vi "Create Synchronized Palette.vi"(6 "Exclude Dir Name pattern":string="^_", 7 "Palette Icon":picture, 8 "error in":errorcluster, 9 "Recursively (F)":bool, 10 "Folder Path":path, 11 "Palette File Path (empty)":path) -> (0 "error out":errorcluster, 2 "All Palette File Paths":path[](array[path]), 3 "Palette File Path out":path)   [LabVIEW 2014, in "VIHelpeksAPI.lvlib"]
doc: "The VI creates a palette file synchronized with the given folder. In addition, if enabled, the VI creates a synchronized palette in every sub-folder beneath the given folder recursively.\n\n<b>Palette icons</b>\nFor the given folder and all sub-folders beneath it (if enabled by <b>Recursively</b>), the VI looks for an image file to use as an icon for the respective palette. A folder's icon file can be one of the following:\n(1) A file with the same name as the folder and a <b>.png</b> extension that resides in the folder's parent directory.\n(2) A file with the <b>dir_icon.png</b> name that resides inside the folder itself.\nIf neither of these icon files is found, a default icon is applied to the respective palette.\nThe icon of the top-level palette can be defined explicitly in the <b>Palette Icon</b> input terminal.\n\n\n::: VI Helpeks :::\nCopyright (c) 2000-2026 Konstantin Shifershteyn. All rights reserved."
uses:
  VIHelpeksAPI.lvlib
  <vilib>/Palette API/Palette Menu/Public Type Define/Palette type.ctl
  <vilib>/Palette API/Palette Menu/Public Type Define/View Format.ctl
  <vilib>/Palette API/Palette Menu/Public Type Define/Palette Data.ctl
  <vilib>/Palette API/Palette Menu/Public Type Define/Items.ctl
  <vilib>/Palette API/Palette Menu/Public Type Define/Item.ctl
  <vilib>/Palette API/Palette Menu/Public Type Define/Help Info.ctl
  <vilib>/Palette API/Palette Menu/Public Type Define/Synchronize Info.ctl
  <vilib>/Palette API/Palette Menu/Palette Menu.lvlib
panel:
  # "VI Helpeks\nCopyright (c) 2012-2026 Konstantin Shifershteyn"
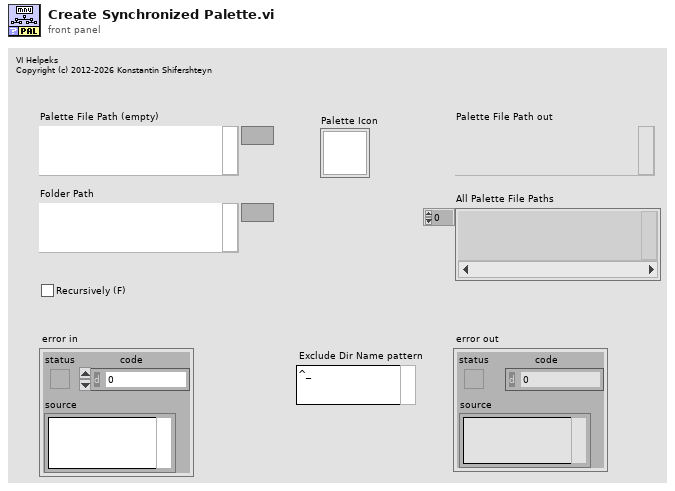
[diagram p1: front panel]
types:
  T1 = typedef "Palette Menu.lvlib/Palette Data.ctl" = cluster{"display name":string, "view format":T2, "palette width":i16, "items":T3, "256 color icon":picture, "B&W color icon":picture, "help information":T5, "palette description":string, "synchronize information":T6}
  T2 = typedef "Palette Menu.lvlib/View Format.ctl" = u16
  T3 = typedef "Palette Menu.lvlib/Items.ctl" = T4[]
  T4 = typedef "Palette Menu.lvlib/Item.ctl" = cluster{"item path":path, "library path (.lvlib)":path, "use default lvlib palette":bool, "short name":string, "place VI contents":bool, "hide synchronized item":bool, "reserve spot for synch item":bool, "configure when placing VI contents":bool}
  T5 = typedef "Palette Menu.lvlib/Help Info.ctl" = cluster{"help tag":string, "help file path ":path}
  T6 = typedef "Palette Menu.lvlib/Synchronize Info.ctl" = cluster{"synchronize with directory":bool, "synchronize directory path":path}
  T7 = typedef "Palette Menu.lvlib/Palette type.ctl" = i32
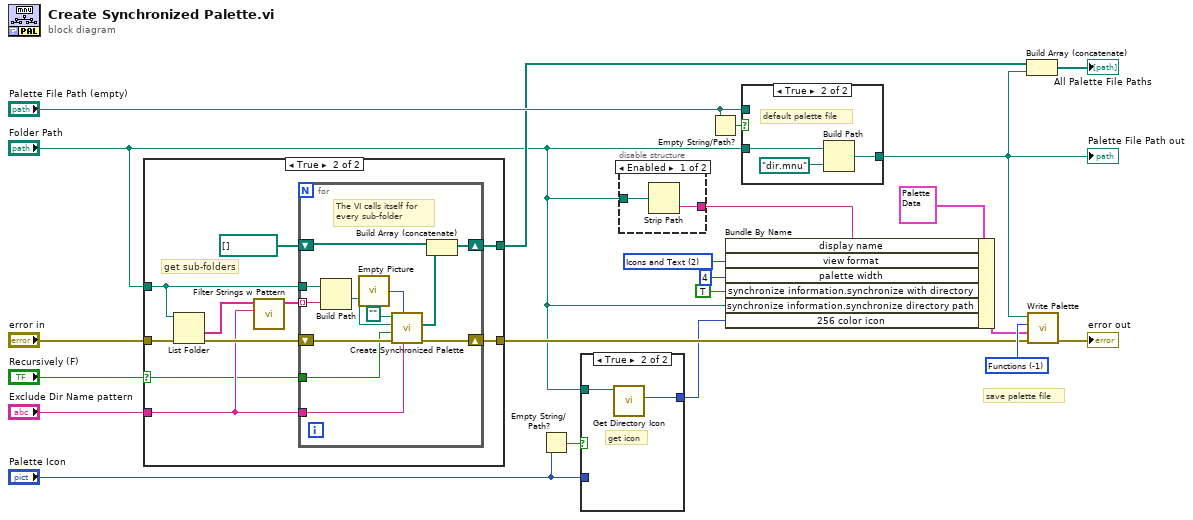
[diagram p0: block diagram]
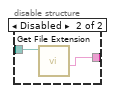
[diagram p5: hidden frame]
diagram:
  w19 = T2 2 items=["Icons", "Text", "Icons and Text"] ("view format")
  w18 = T7 -1 items=["Functions"=-1, "Controls"=-2] ("palette type")
  # "save palette file"
  n1 = case shown="True" "Recursively (F)" {
    selector: "Recursively (F)" -> [_ w25]
    tunnel: "error in" -> [w22 w32]
    tunnel: [w22 w29] -> w15
    tunnel: "Exclude Dir Name pattern" -> [_ w26]
    tunnel: "Folder Path" -> [_ w27]
    tunnel: [_ w23] -> w7
    frame False {
    }
    frame True {
      # "get sub-folders"
      n2 = List Folder(path=w27, error in=w32) -> (folder names=w31:string[], error out=w30:errorcluster)  [unwired: 2 in, 2 out]
      n3 = call "Filter Strings w Pattern.vi"("Exclude pattern(s) (^_)"=w26, "Array in"=w31) -> ("Array out"=w28:string[])  [unwired: 9 in]
      n4 = for {
        tunnel: w27 -> [w44]
        tunnel: w28 -> [w41] mode=indexing
        shift-right: [w42] -> w29
        shift-left: w30 -> [w43]
        tunnel: w26 -> [w40]
        tunnel: w25 -> [w39]
        shift-right: [w34] -> w23
        shift-left: path[] [] -> [w35]
        # "The VI calls itself for\nevery sub-folder"
        n5 = Build Path(base path=w44, name or relative path=w41) -> (appended path=w38:path)
        n6 = call "Empty Picture"() -> ("empty picture"=w33:picture)
        n7 = call "Create Synchronized Palette.vi"("Exclude Dir Name pattern"=w40, "Palette Icon"=w33, "error in"=w43, "Recursively (F)"=w39, "Folder Path"=w38, "Palette File Path (empty)"=path "") -> ("error out"=w42:errorcluster, "All Palette File Paths"=w36:path[])  [unwired: 3 in, 1 out]
        n8 = Build Array (concatenate)(w35, w36) -> (w34:path[])
      }
    }
  }
  n9 = Empty String/Path?(string/path="Palette Icon") -> (empty?=w3:bool)
  n10 = case shown="True" w3 {
    tunnel: [w45 w47] -> w1
    tunnel: "Folder Path" -> [_ w46]
    tunnel: "Palette Icon" -> [w45 _]
    frame False {
    }
    frame True {
      # "get icon"
      n11 = call "Get Directory Icon.vi"("Directory Path"=w46) -> ("Icon"=w47:picture)  [unwired: 8 in, 2 out]
    }
  }
  n12 = disable-structure shown="Enabled" {
    disable-tunnel: "Folder Path" -> [w49 w51]
    disable-tunnel: [w48 w50] -> w20
    frame Enabled {
      n13 = Strip Path(path=w49) -> (name=w48:string)  [unwired: 1 out]
    }
    frame Disabled {
      n14 = call <vilib>:"Get File Extension.vi"("file"=w51) -> ("filename without extension"=w50:string)  [unwired: 7 in, 3 out]
    }
  }
  n15 = Empty String/Path?(string/path="Palette File Path (empty)") -> (empty?=w9:bool)
  n16 = Bundle By Name(cluster=T1 {"display name"="", "view format"=2, "palette width"=4, "items"=[], "256 color icon"=bytes[0], "B&W color icon"=bytes[0], "help information"={"help tag"="", "help file path "=path ""}, "palette description"="", "synchronize information"={"synchronize with directory"=FALSE, "synchronize directory path"=path ""}} ("palette data"), "display name"=w20, "view format"=w19, "palette width"=i16 4, "synchronize information.synchronize with directory"=TRUE, "synchronize information.synchronize directory path"="Folder Path", "256 color icon"=w1) -> (w17:T1)
  n17 = case shown="True" w9 {
    tunnel: [w52 w54] -> w6
    tunnel: "Folder Path" -> [_ w53]
    tunnel: "Palette File Path (empty)" -> [w52 _]
    frame False {
    }
    frame True {
      # "default palette file"
      n18 = Build Path(base path=w53, name or relative path=path "dir.mnu") -> (appended path=w54:path)
    }
  }
  "Palette File Path out" <- w6
  n19 = Build Array (concatenate)(w7, w6) -> (→"All Palette File Paths":path[])
  n20 = call <vilib>:"Write Palette.vi"("error in (no error)"=w15, "palette data"=w17, "palette type"=w18, "palette path"=w6) -> ("error out"=→"error out":errorcluster)  [unwired: 7 in]
